vi "set BW and DL Channel Number.vi"(8 "error in (no error)":errorcluster caption="에러 입력(에러 없음)", 9 "PCC Downlink":i32, 10 "BandWidth":T1, 11 "LTE 입력":refnum<class "LTE.lvclass">) -> (0 "error out":errorcluster caption="에러 출력", 3 "LTE 출력":refnum<class "LTE.lvclass">)   [LabVIEW 2023, in "ANRITSU Call Box.lvlib" / "LTE.lvclass"]
uses:
  LTE.lvclass
  Type Definition/LTE Supported BandWidth.ctl
  LTE.lvclass/LTE.ctl
  ANRITSU Call Box.lvlib
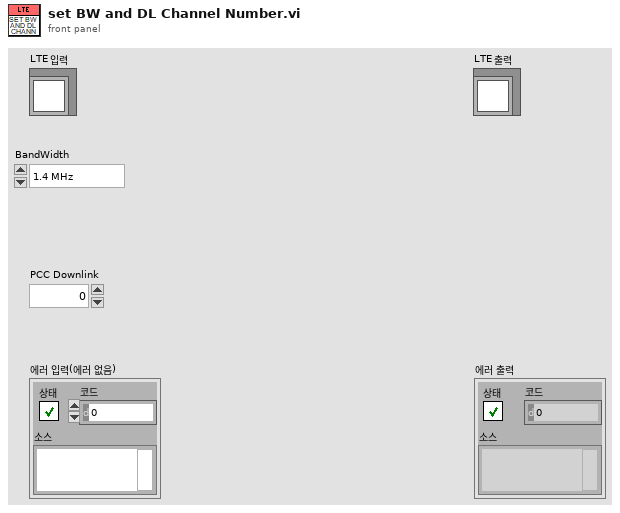
[diagram p1: front panel]
types:
  T1 = typedef "ANRITSU Call Box.lvlib/LTE Supported BandWidth.ctl" = enum16{"1.4 MHz", "3 MHz", "5 MHz", "10 MHz", "15 MHz", "20 MHz"}
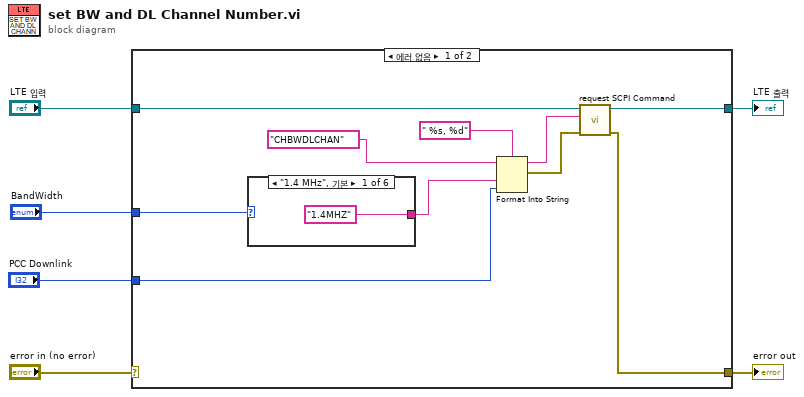
[diagram p0: block diagram]
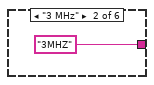
[diagram p2: hidden frame]
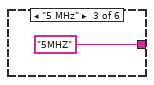
[diagram p3: hidden frame]
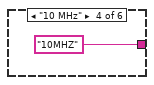
[diagram p4: hidden frame]
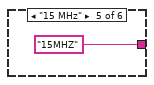
[diagram p5: hidden frame]
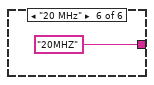
[diagram p6: hidden frame]
diagram:
  n1 = case shown="에러 없음" "error in (no error)" {
    selector: "error in (no error)" -> [_ w24]
    tunnel: [w11 w24] -> w5
    tunnel: [w15 w23] -> w3
    tunnel: "LTE 입력" -> [w16 w23]
    tunnel: "BandWidth" -> [w13 _]
    tunnel: "PCC Downlink" -> [w8 _]
    frame No Error {
      n2 = case shown="\"1.4 MHz\", 기본" w13 {
        tunnel: ["1.4MHZ" "3MHZ" "5MHZ" "10MHZ" "15MHZ" "20MHZ"] -> w9
        frame "1.4 MHz", Default {
        }
        frame "3 MHz" {
        }
        frame "5 MHz" {
        }
        frame "10 MHz" {
        }
        frame "15 MHz" {
        }
        frame "20 MHz" {
        }
      }
      n3 = Format Into String(format string=" %s, %d", initial string="CHBWDLCHAN" ("string"), w9, w8) -> (resulting string=w7:string, error out=w12:errorcluster)  [unwired: 1 in]
      n4 = call "request SCPI Command.vi"("error in (no error)"=w12, "SCPI Command"=w7, "LTE in"=w16) -> ("error out"=w11:errorcluster, "LTE out"=w15:refnum<class "LTE.lvclass">)  [unwired: 7 in]
    }
    frame Error {
    }
  }
  "error out" <- w5
  "LTE 출력" <- w3
